vi "Mem.vi"() -> ()   [LabVIEW 2020]
doc: "Dev helper: names of the VIs in memory (main instance) that contain text, comma-joined."
panel:
  out "names":string
  in  "text":string="RemoteVI"
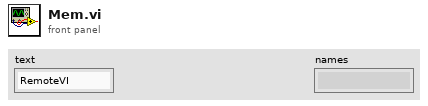
[diagram p1: front panel]
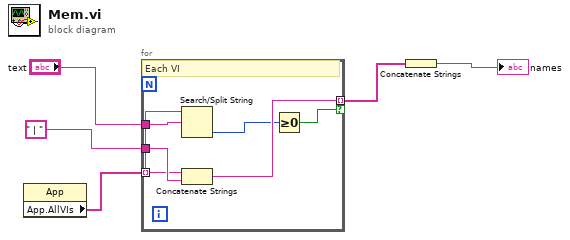
[diagram p0: block diagram]
diagram:
  n1 = property class="App"() -> ("App.AllVIs"=w2:string[])  [unwired: 2 in, 2 out]
  n2 = for {
    tunnel: "text" -> [w7]
    tunnel: " | " -> [w8]
    tunnel: w2 -> [w6] mode=indexing
    tunnel: [w11] -> w4 mode=indexing if=w10
    # "Each VI"
    n3 = Search/Split String(string=w6, search string/char (-)=w7) -> (offset of match=w9:i32)  [unwired: 1 in, 2 out]
    n4 = Concatenate Strings(w6, w8) -> (w11:string)
    n5 = Greater Or Equal To 0?(x=w9) -> (x >= 0?=w10:bool)
  }
  n6 = Concatenate Strings(w4) -> (→"names":string)
